vi "Set Value of LabVIEW Base Type.vi"(8 "error in (no error)":errorcluster, 10 "LabVIEW Base Type":refnum<vi>, 11 "JSON Tree Node":variant) -> (0 "error out":errorcluster)   [LabVIEW 2014, in "i3-json.lvlib"]
doc: "This VI takes a JSON Node (all types besides JSON Object) and assigns the value to the LabVIEW Base Type of compatible reference.\n\nIf the LabVIEW base type is an array of boolean, numeric, or string this function will attempt to check if a JSON Array type will map"
uses:
  i3-json.lvlib
  JSON Types/JSON Type.ctl
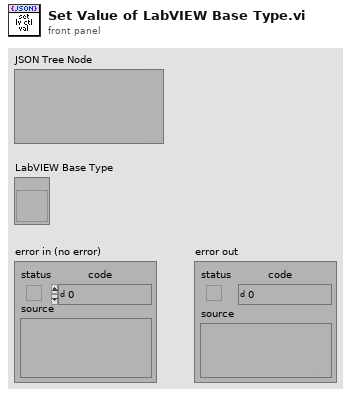
[diagram p1: front panel]
types:
  T1 = typedef "i3-json.lvlib/JSON Type.ctl" = enum8{"JSON Compatible", "JSON Array", "JSON Object", "JSON Null", "Double", "String", "Boolean", "Unknown"}
  T2 = enum8{"Invalid Type", "Void", "I8", "I16", "I32", "I64", "U8", "U16", "U32", "U64", "Single Float", "Double Float", "Extended Float", "Single Complex", "Double Complex", "Extended Complex", "Enum U8", "Enum U16", "Enum U32", "Enum U64", "Single Float With Unit", "Double Float With Unit", "Extended Float With Unit", "Single Complex with Unit", "Double Complex with Unit", "Extended Complex with Unit", "Boolean", "String", "Path", "Picture", "Tag", "Array", "Cluster", "Variant", "LV Variant", "Waveform", "Timestamp", "Digital Waveform", "Digital Data", "ExpressData", "Refnum", "External Data", "VI", "Poly VI", "LabVIEW Class Instance", "Fixed Point"}
  T3 = typedef "i3-json.lvlib/JSON Compatible Type.ctl" = enum16{"1D Double Array", "1D String Array", "1D Boolean Array", "Unknown"}
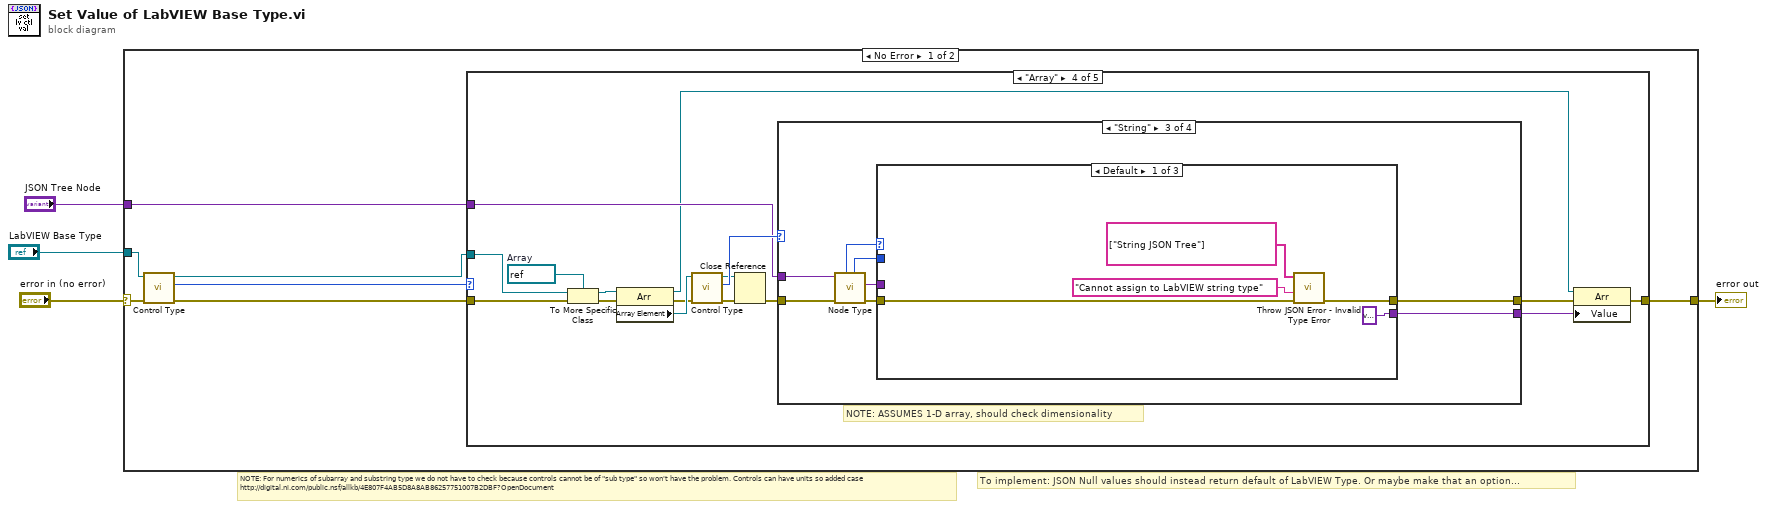
[diagram p0: block diagram]
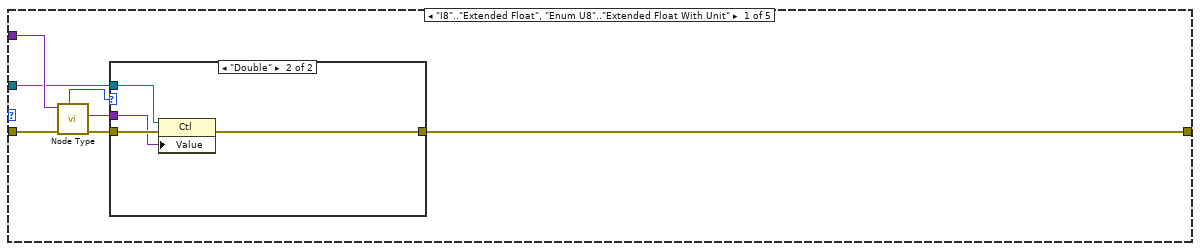
[diagram p2: hidden frame]
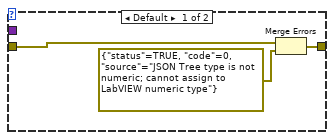
[diagram p3: hidden frame]
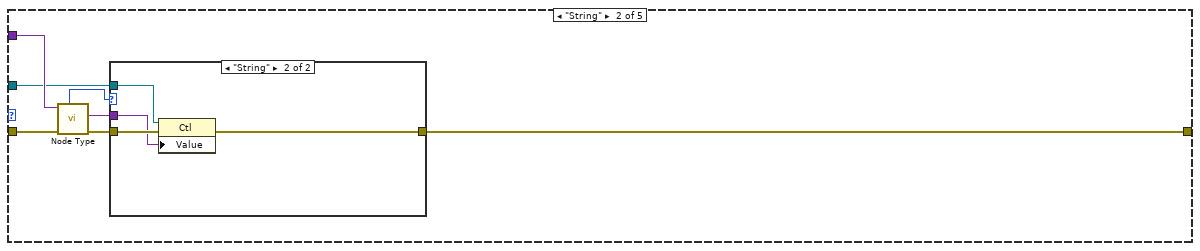
[diagram p4: hidden frame]
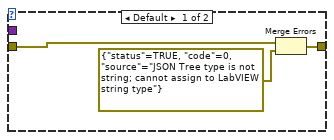
[diagram p5: hidden frame]
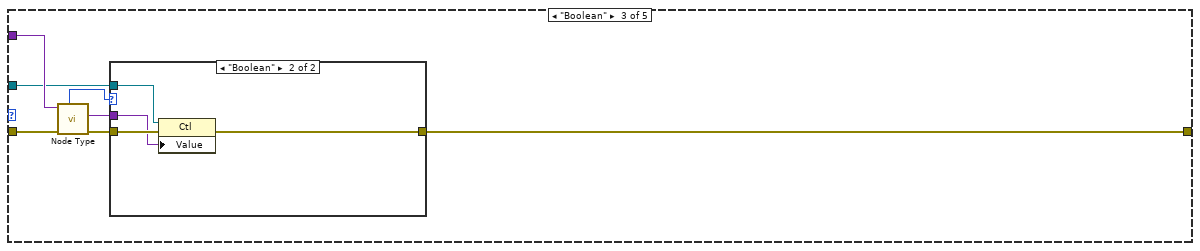
[diagram p6: hidden frame]
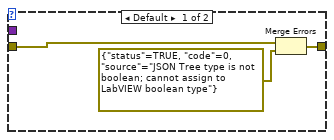
[diagram p7: hidden frame]
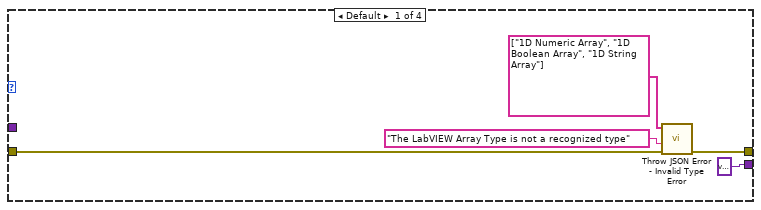
[diagram p8: hidden frame]
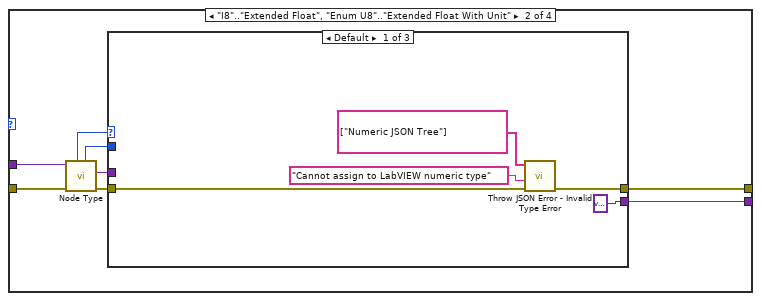
[diagram p9: hidden frame]
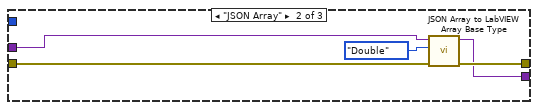
[diagram p10: hidden frame]
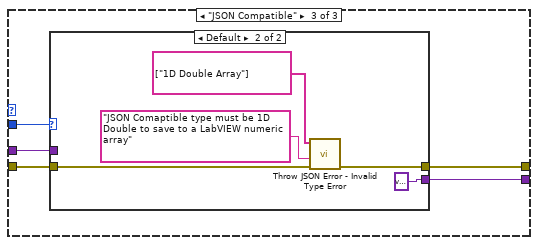
[diagram p11: hidden frame]
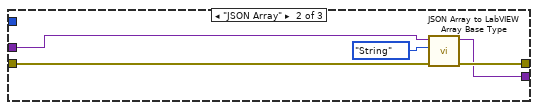
[diagram p13: hidden frame]
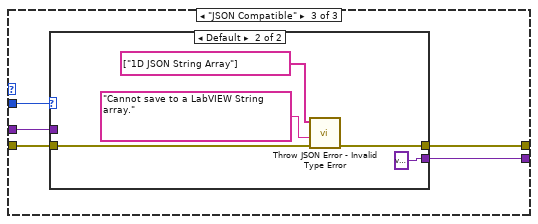
[diagram p14: hidden frame]
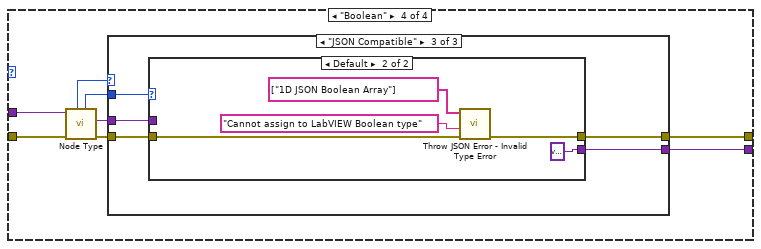
[diagram p16: hidden frame]
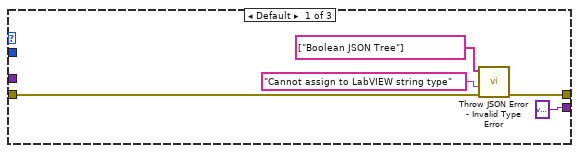
[diagram p17: hidden frame]
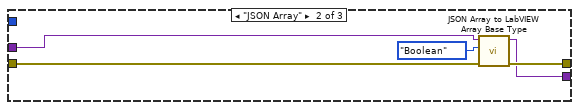
[diagram p18: hidden frame]
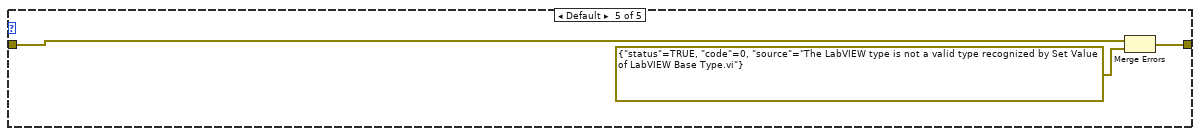
[diagram p20: hidden frame]
diagram:
  # "NOTE: For numerics of subarray and substring type we do not have to check because controls cannot be of \"sub type\" so won't have the problem. Controls can have units so added case\nhttp://digital.ni.com/public.nsf/allkb/4E807F4AB5D8A8AB86257751007B2DBF?OpenDocument"
  # "To implement: JSON Null values should instead return default of LabVIEW Type. Or maybe make that an option..."
  n1 = case shown="No Error" "error in (no error)" {
    selector: "error in (no error)" -> [w11 w168]
    tunnel: "LabVIEW Base Type" -> [w10 _]
    tunnel: "JSON Tree Node" -> [w7 _]
    tunnel: [w5 w168] -> w1
    frame No Error {
      n2 = call "Control Type.vi"("error in (no error)"=w11, "Control in"=w10) -> ("error out"=w6:errorcluster, "Type"=w9:T2, "Control out"=w8:refnum<vi>)  [unwired: 7 in]
      n3 = case shown="\"Array\"" w9 {
        tunnel: w8 -> [w13 w27 w41 w68 _]
        tunnel: w7 -> [w18 w32 w46 w63 _]
        tunnel: w6 -> [w17 w31 w45 w69 w167]
        tunnel: [w12 w26 w40 w60 w166] -> w5
        frame "I8".."Extended Float", "Enum U8".."Extended Float With Unit" {
          n4 = call "Node Type.vi"("error in (no error)"=w17, "JSON Tree In"=w18) -> ("error out"=w15:errorcluster, "Value"=w14:variant, "JSON Type"=w16:T1)  [unwired: 5 in, 2 out]
          n5 = case shown="\"Double\"" w16 {
            tunnel: w15 -> [w21 w25]
            tunnel: [w19 w22] -> w12
            tunnel: w14 -> [_ w24]
            tunnel: w13 -> [_ w23]
            frame Default {
              n6 = Merge Errors(w21, errorcluster {"status"=TRUE, "code"=0, "source"="JSON Tree type is not numeric; cannot assign to LabVIEW numeric type"} ("error in")) -> (w19:errorcluster)
            }
            frame "Double" {
              n7 = property class="Ctl"(reference=w23, error in=w25, "Value"=w24) -> (error out=w22:errorcluster)  [unwired: 1 out]
            }
          }
        }
        frame "String" {
          n8 = call "Node Type.vi"("error in (no error)"=w31, "JSON Tree In"=w32) -> ("error out"=w29:errorcluster, "Value"=w28:variant, "JSON Type"=w30:T1)  [unwired: 5 in, 2 out]
          n9 = case shown="\"String\"" w30 {
            tunnel: w29 -> [w35 w39]
            tunnel: [w33 w36] -> w26
            tunnel: w28 -> [_ w38]
            tunnel: w27 -> [_ w37]
            frame Default {
              n10 = Merge Errors(w35, errorcluster {"status"=TRUE, "code"=0, "source"="JSON Tree type is not string; cannot assign to LabVIEW string type"} ("error in")) -> (w33:errorcluster)
            }
            frame "String" {
              n11 = property class="Ctl"(reference=w37, error in=w39, "Value"=w38) -> (error out=w36:errorcluster)  [unwired: 1 out]
            }
          }
        }
        frame "Boolean" {
          n12 = call "Node Type.vi"("error in (no error)"=w45, "JSON Tree In"=w46) -> ("error out"=w43:errorcluster, "Value"=w42:variant, "JSON Type"=w44:T1)  [unwired: 5 in, 2 out]
          n13 = case shown="\"Boolean\"" w44 {
            tunnel: w43 -> [w49 w53]
            tunnel: [w47 w50] -> w40
            tunnel: w42 -> [_ w52]
            tunnel: w41 -> [_ w51]
            frame Default {
              n14 = Merge Errors(w49, errorcluster {"status"=TRUE, "code"=0, "source"="JSON Tree type is not boolean; cannot assign to LabVIEW boolean type"} ("error in")) -> (w47:errorcluster)
            }
            frame "Boolean" {
              n15 = property class="Ctl"(reference=w51, error in=w53, "Value"=w52) -> (error out=w50:errorcluster)  [unwired: 1 out]
            }
          }
        }
        frame "Array" {
          w62 = refnum<vi> refnum  # Array
          # "NOTE: ASSUMES 1-D array, should check dimensionality"
          n16 = To More Specific Class(target class=w62, reference=w68, error in=w69) -> (specific class reference=w59:refnum<vi>, error out=w67:errorcluster)
          n17 = property class="Arr"(reference=w59, error in=w67) -> (reference out=w54:refnum<vi>, error out=w65:errorcluster, "Array Element"=w66:refnum<vi>)
          n18 = call "Control Type.vi"("error in (no error)"=w65, "Control in"=w66) -> ("error out"=w57:errorcluster, "Type"=w64:T2, "Control out"=w55:refnum<vi>)  [unwired: 7 in]
          n19 = Close Reference(reference=w55, error in (no error)=w57) -> (error out=w56:errorcluster)
          n20 = case shown="\"String\"" w64 {
            tunnel: w56 -> [w73 w80 w110 w140]
            tunnel: w63 -> [_ w79 w109 w139]
            tunnel: [w72 w76 w106 w136] -> w61
            tunnel: [variant ("Value") w75 w105 w135] -> w58
            frame Default {
              n21 = call "Throw JSON Error - Invalid Type Error.vi"("error in (no error)"=w73, "additional info"="The LabVIEW Array Type is not a recognized type" ("source"), "Valid Types"=string[] ["1D Numeric Array", "1D Boolean Array", "1D String Array"]) -> ("error out"=w72:errorcluster)  [unwired: 8 in]
            }
            frame "I8".."Extended Float", "Enum U8".."Extended Float With Unit" {
              n22 = call "Node Type.vi"("error in (no error)"=w80, "JSON Tree In"=w79) -> ("error out"=w81:errorcluster, "Value"=w82:variant, "JSON Compatible Type"=w77:T3, "JSON Type"=w78:T1)  [unwired: 5 in, 1 out]
              n23 = case shown="Default" w78 {
                tunnel: w81 -> [w86 w92 w96]
                tunnel: w82 -> [_ w91 w95]
                tunnel: [w85 w89 w97] -> w76
                tunnel: w77 -> [_ _ w94]
                tunnel: [variant ("Value") w88 w93] -> w75
                frame Default {
                  n24 = call "Throw JSON Error - Invalid Type Error.vi"("error in (no error)"=w86, "additional info"="Cannot assign to LabVIEW numeric type" ("source"), "Valid Types"=string[] ["Numeric JSON Tree"]) -> ("error out"=w85:errorcluster)  [unwired: 8 in]
                }
                frame "JSON Array" {
                  n25 = call "JSON Array to LabVIEW Array Base Type.vi"("error in (no error)"=w92, "Type of Array In"=JSON_Type."Double", "JSON Array In"=w91) -> ("error out"=w89:errorcluster, "LabVIEW Array Base Type Out"=w88:variant)  [unwired: 7 in]
                }
                frame "JSON Compatible" {
                  n26 = case shown="Default" w94 {
                    tunnel: w96 -> [w98 w101]
                    tunnel: [w98 w100] -> w97
                    tunnel: w95 -> [w99 _]
                    tunnel: [w99 variant ("Value")] -> w93
                    frame "1D Double Array" {
                    }
                    frame Default {
                      n27 = call "Throw JSON Error - Invalid Type Error.vi"("error in (no error)"=w101, "additional info"="JSON Comaptible type must be 1D Double to save to a LabVIEW numeric array" ("source"), "Valid Types"=string[] ["1D Double Array"]) -> ("error out"=w100:errorcluster)  [unwired: 8 in]
                    }
                  }
                }
              }
            }
            frame "String" {
              n28 = call "Node Type.vi"("error in (no error)"=w110, "JSON Tree In"=w109) -> ("error out"=w111:errorcluster, "Value"=w112:variant, "JSON Compatible Type"=w107:T3, "JSON Type"=w108:T1)  [unwired: 5 in, 1 out]
              n29 = case shown="Default" w108 {
                tunnel: w111 -> [w116 w122 w126]
                tunnel: w112 -> [_ w121 w125]
                tunnel: [w115 w119 w127] -> w106
                tunnel: w107 -> [_ _ w124]
                tunnel: [variant ("Value") w118 w123] -> w105
                frame Default {
                  n30 = call "Throw JSON Error - Invalid Type Error.vi"("error in (no error)"=w116, "additional info"="Cannot assign to LabVIEW string type" ("source"), "Valid Types"=string[] ["String JSON Tree"]) -> ("error out"=w115:errorcluster)  [unwired: 8 in]
                }
                frame "JSON Array" {
                  n31 = call "JSON Array to LabVIEW Array Base Type.vi"("error in (no error)"=w122, "Type of Array In"=JSON_Type."String", "JSON Array In"=w121) -> ("error out"=w119:errorcluster, "LabVIEW Array Base Type Out"=w118:variant)  [unwired: 7 in]
                }
                frame "JSON Compatible" {
                  n32 = case shown="Default" w124 {
                    tunnel: w126 -> [w128 w131]
                    tunnel: [w128 w130] -> w127
                    tunnel: w125 -> [w129 _]
                    tunnel: [w129 variant ("Value")] -> w123
                    frame "1D String Array" {
                    }
                    frame Default {
                      n33 = call "Throw JSON Error - Invalid Type Error.vi"("error in (no error)"=w131, "additional info"="Cannot save to a LabVIEW String array." ("source"), "Valid Types"=string[] ["1D JSON String Array"]) -> ("error out"=w130:errorcluster)  [unwired: 8 in]
                    }
                  }
                }
              }
            }
            frame "Boolean" {
              n34 = call "Node Type.vi"("error in (no error)"=w140, "JSON Tree In"=w139) -> ("error out"=w141:errorcluster, "Value"=w142:variant, "JSON Compatible Type"=w137:T3, "JSON Type"=w138:T1)  [unwired: 5 in, 1 out]
              n35 = case shown="\"JSON Compatible\"" w138 {
                tunnel: w141 -> [w144 w152 w156]
                tunnel: w142 -> [_ w151 w155]
                tunnel: [w143 w149 w157] -> w136
                tunnel: w137 -> [_ _ w154]
                tunnel: [variant ("Value") w148 w153] -> w135
                frame Default {
                  n36 = call "Throw JSON Error - Invalid Type Error.vi"("error in (no error)"=w144, "additional info"="Cannot assign to LabVIEW string type" ("source"), "Valid Types"=string[] ["Boolean JSON Tree"]) -> ("error out"=w143:errorcluster)  [unwired: 8 in]
                }
                frame "JSON Array" {
                  n37 = call "JSON Array to LabVIEW Array Base Type.vi"("error in (no error)"=w152, "Type of Array In"=JSON_Type."Boolean", "JSON Array In"=w151) -> ("error out"=w149:errorcluster, "LabVIEW Array Base Type Out"=w148:variant)  [unwired: 7 in]
                }
                frame "JSON Compatible" {
                  n38 = case shown="Default" w154 {
                    tunnel: w156 -> [w158 w160]
                    tunnel: [w158 w161] -> w157
                    tunnel: w155 -> [w159 _]
                    tunnel: [w159 variant ("Value")] -> w153
                    frame "1D Boolean Array" {
                    }
                    frame Default {
                      n39 = call "Throw JSON Error - Invalid Type Error.vi"("error in (no error)"=w160, "additional info"="Cannot assign to LabVIEW Boolean type" ("source"), "Valid Types"=string[] ["1D JSON Boolean Array"]) -> ("error out"=w161:errorcluster)  [unwired: 8 in]
                    }
                  }
                }
              }
            }
          }
          n40 = property class="Arr"(reference=w54, error in=w61, "Value"=w58) -> (error out=w60:errorcluster)  [unwired: 1 out]
        }
        frame Default {
          n41 = Merge Errors(w167, errorcluster {"status"=TRUE, "code"=0, "source"="The LabVIEW type is not a valid type recognized by Set Value of LabVIEW Base Type.vi"} ("error in")) -> (w166:errorcluster)
        }
      }
    }
    frame Error {
    }
  }
  "error out" <- w1
